vi "Nouvelles donnees.vi"(0 "Nb Capteurs":i32, 1 "offset entrée (en octets) (0)":i64) -> (2 "Nouvelles données":string[](array[string]), 3 "Nouveau temps":dbl, 4 "Chemin du fichier local :":path, 5 "offset sortie (en octets)":i64)   [LabVIEW 2022 SP3]
uses:
  Variables globales/Variable glob generale.vi
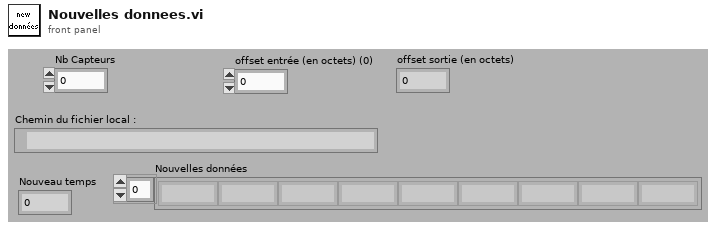
[diagram p1: front panel]
types:
  T1 = enum16{"open", "replace", "create", "open or create", "replace or create", "replace or create with confirmation"}
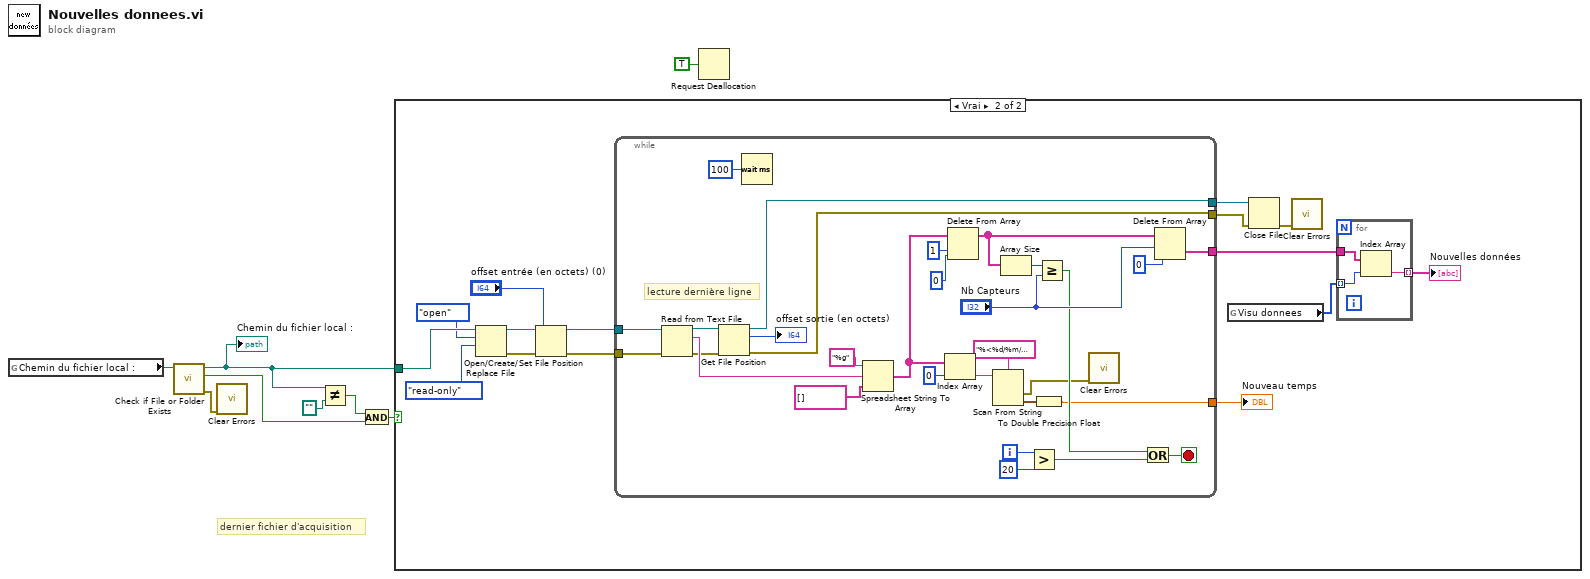
[diagram p0: block diagram]
diagram:
  # "dernier fichier d'acquisition"
  n1 = global read "Variable glob generale.vi" "Chemin du fichier local :"() -> (w6:path)
  n2 = call <vilib>:"Check if File or Folder Exists.vi"("path"=w6) -> ("error out"=w4:errorcluster, "file or folder exists?"=w2:bool, "dup path"=w5:path)  [unwired: 8 in]
  "Chemin du fichier local :" <- w5
  n3 = call <vilib>:"Clear Errors.vi"("error in (no error)"=w4) -> ()  [unwired: 5 in, 2 out]
  n4 = Not Equal?(x=w5, y=path "") -> (x != y?=w3:bool)
  n5 = And(x=w3, y=w2) -> (x .and. y?=w1:bool)
  n6 = case shown="Vrai" w1 {
    tunnel: w5 -> [_ w19]
    frame False {
    }
    frame True {
      n7 = Open/Create/Replace File(file path (use dialog)=w19, operation (0:open)=T1."open" ("opération (0 : open)"), access (0:read/write)=enum16{"read/write", "read-only", "write-only"}."read-only" ("accès (0 : read/write)")) -> (refnum out=w16:refnum<file>, error out=w15:errorcluster)  [unwired: 3 in, 1 out]
      n8 = Set File Position(offset (in bytes) (0)="offset entrée (en octets) (0)", refnum=w16, error in=w15) -> (refnum out=w13:refnum<file>, error out=w11:errorcluster)  [unwired: 1 in]
      n9 = while {
        tunnel: [w56] -> w21
        tunnel: [w28] -> w23
        tunnel: w13 -> [w39]
        tunnel: [w35] -> w12
        tunnel: w11 -> [w34]
        tunnel: [w32] -> w10
        i -> [w48]
        stop <- w44 stop-if-true
        # "lecture dernière ligne"
        n10 = Read from Text File(file (use dialog)=w39, error in=w34) -> (refnum out=w38:refnum<file>, text=w37:string, error out=w33:errorcluster)  [unwired: 2 in, 1 out]
        n11 = Get File Position(4:w33, 7:w38) -> (0:w32:errorcluster, 2:→"offset sortie (en octets)":i64, 3:w35:refnum<file>)
        n12 = Wait (ms)(milliseconds to wait=u32 100 ("attente (ms)")) -> ()  [unwired: 1 out]
        n13 = Spreadsheet String To Array(format string="%g" ("chaîne de format"), spreadsheet string=w37, array type (2D Dbl)=string[] [] ("type de tableau (2D de dbl)")) -> (array=w49:string[])  [unwired: 1 in]
        n14 = Index Array(array=w49, index=0 ("indice")) -> (element=w29:string)
        n15 = Delete From Array(array=w49, length=1 ("longueur"), index=0 ("indice")) -> (array with subset deleted=w43:string[])  [unwired: 1 out]
        n16 = Scan From String(format string="%<%d/%m/%Y%2u%H:%M:%S>T" ("chaîne de format"), input string=w29) -> (error out=w27:errorcluster, output 1=w30:timestamp)  [unwired: 3 in, 2 out]
        n17 = Array Size(array=w43) -> (size(s)=w42:i32)
        n18 = Greater?(x=w48, y=20) -> (0:w45:bool)
        n19 = To Double Precision Float(number=w30) -> (double precision float=w28:dbl)
        n20 = Greater Or Equal?(x=w42, y="Nb Capteurs") -> (x >= y?=w40:bool)
        n21 = call <vilib>:"Clear Errors.vi"("error in (no error)"=w27) -> ()  [unwired: 5 in, 2 out]
        n22 = Or(x=w40, y=w45) -> (x .or. y?=w44:bool)
        n23 = Delete From Array(array=w43, length="Nb Capteurs", index=0 ("indice")) -> (deleted portion=w56:string[])  [unwired: 1 out]
      }
      "Nouveau temps" <- w23
      n24 = global read "Variable glob generale.vi" "Visu donnees"() -> (w22:i32[])
      n25 = Close File(refnum=w12, error in=w10) -> (error out=w9:errorcluster)  [unwired: 1 out]
      n26 = call <vilib>:"Clear Errors.vi"("error in (no error)"=w9) -> ()  [unwired: 5 in, 2 out]
      n27 = for {
        tunnel: w22 -> [w25] mode=indexing
        tunnel: w21 -> [w26]
        tunnel: [w24] -> w20 mode=indexing
        n28 = Index Array(array=w26, index=w25) -> (element=w24:string)
      }
      "Nouvelles données" <- w20
    }
  }
  n29 = Request Deallocation(TRUE ("flag")) -> ()
